vi "BaseProvider_DesignPattern_GetPatterns.vi"(1 "FilterOnProviders(Ignored If Empty)":string, 2 "FilterOnTemplate(Ignored If Empty)":string, 5 "error in (no error)":errorcluster) -> (15 "DesignPatterns":T1[](array[typedef]), 19 "error out":errorcluster)   [LabVIEW 2020]
uses:
  DesignPatternsData.ctl
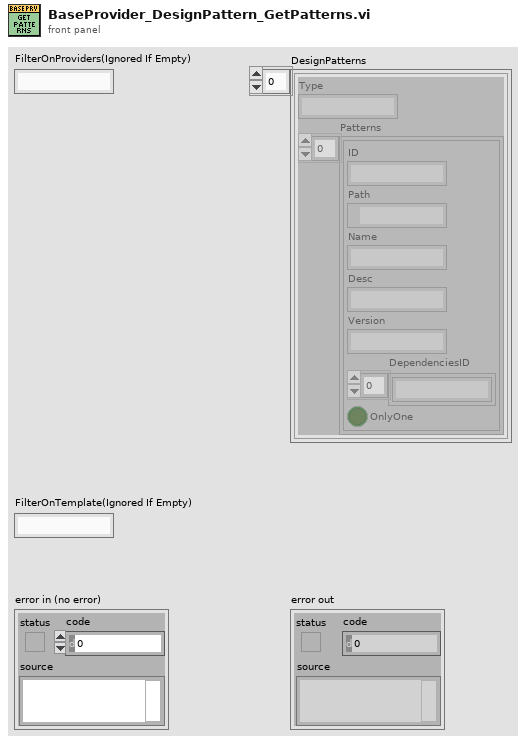
[diagram p1: front panel]
types:
  T1 = typedef "DesignPatternsData.ctl" = cluster{"Type":string, "Patterns":cluster{"ID":string, "Path":path, "Name":string, "Desc":string, "Version":string, "DependenciesID":string[], "OnlyOne":bool}[]}
  T2 = cluster{"Cancelled":bool, "IniFiles":path[], "IniFilesContent":cluster{"ID":string, "Version":string, "PlugIn":path, "Type":string, "Name":string, "Desc":string, "Supports":cluster{"Provider":string, "Templates":string}[], "DependenciesID":string[], "OnlyOne":bool}[], "DesignPatterns":T1[]}
  T3 = cluster{"ID":string, "Version":string, "PlugIn":path, "Type":string, "Name":string, "Desc":string, "Supports":cluster{"Provider":string, "Templates":string}[], "DependenciesID":string[], "OnlyOne":bool}[]
  T4 = cluster{"ID":string, "Version":string, "PlugIn":path, "Type":string, "Name":string, "Desc":string, "Supports":cluster{"Provider":string, "Templates":string}[], "DependenciesID":string[], "OnlyOne":bool}
  T5 = cluster{"ID":string, "Path":path, "Name":string, "Desc":string, "Version":string, "DependenciesID":string[], "OnlyOne":bool}[]
  T6 = cluster{"ID":string, "Path":path, "Name":string, "Desc":string, "Version":string, "DependenciesID":string[], "OnlyOne":bool}
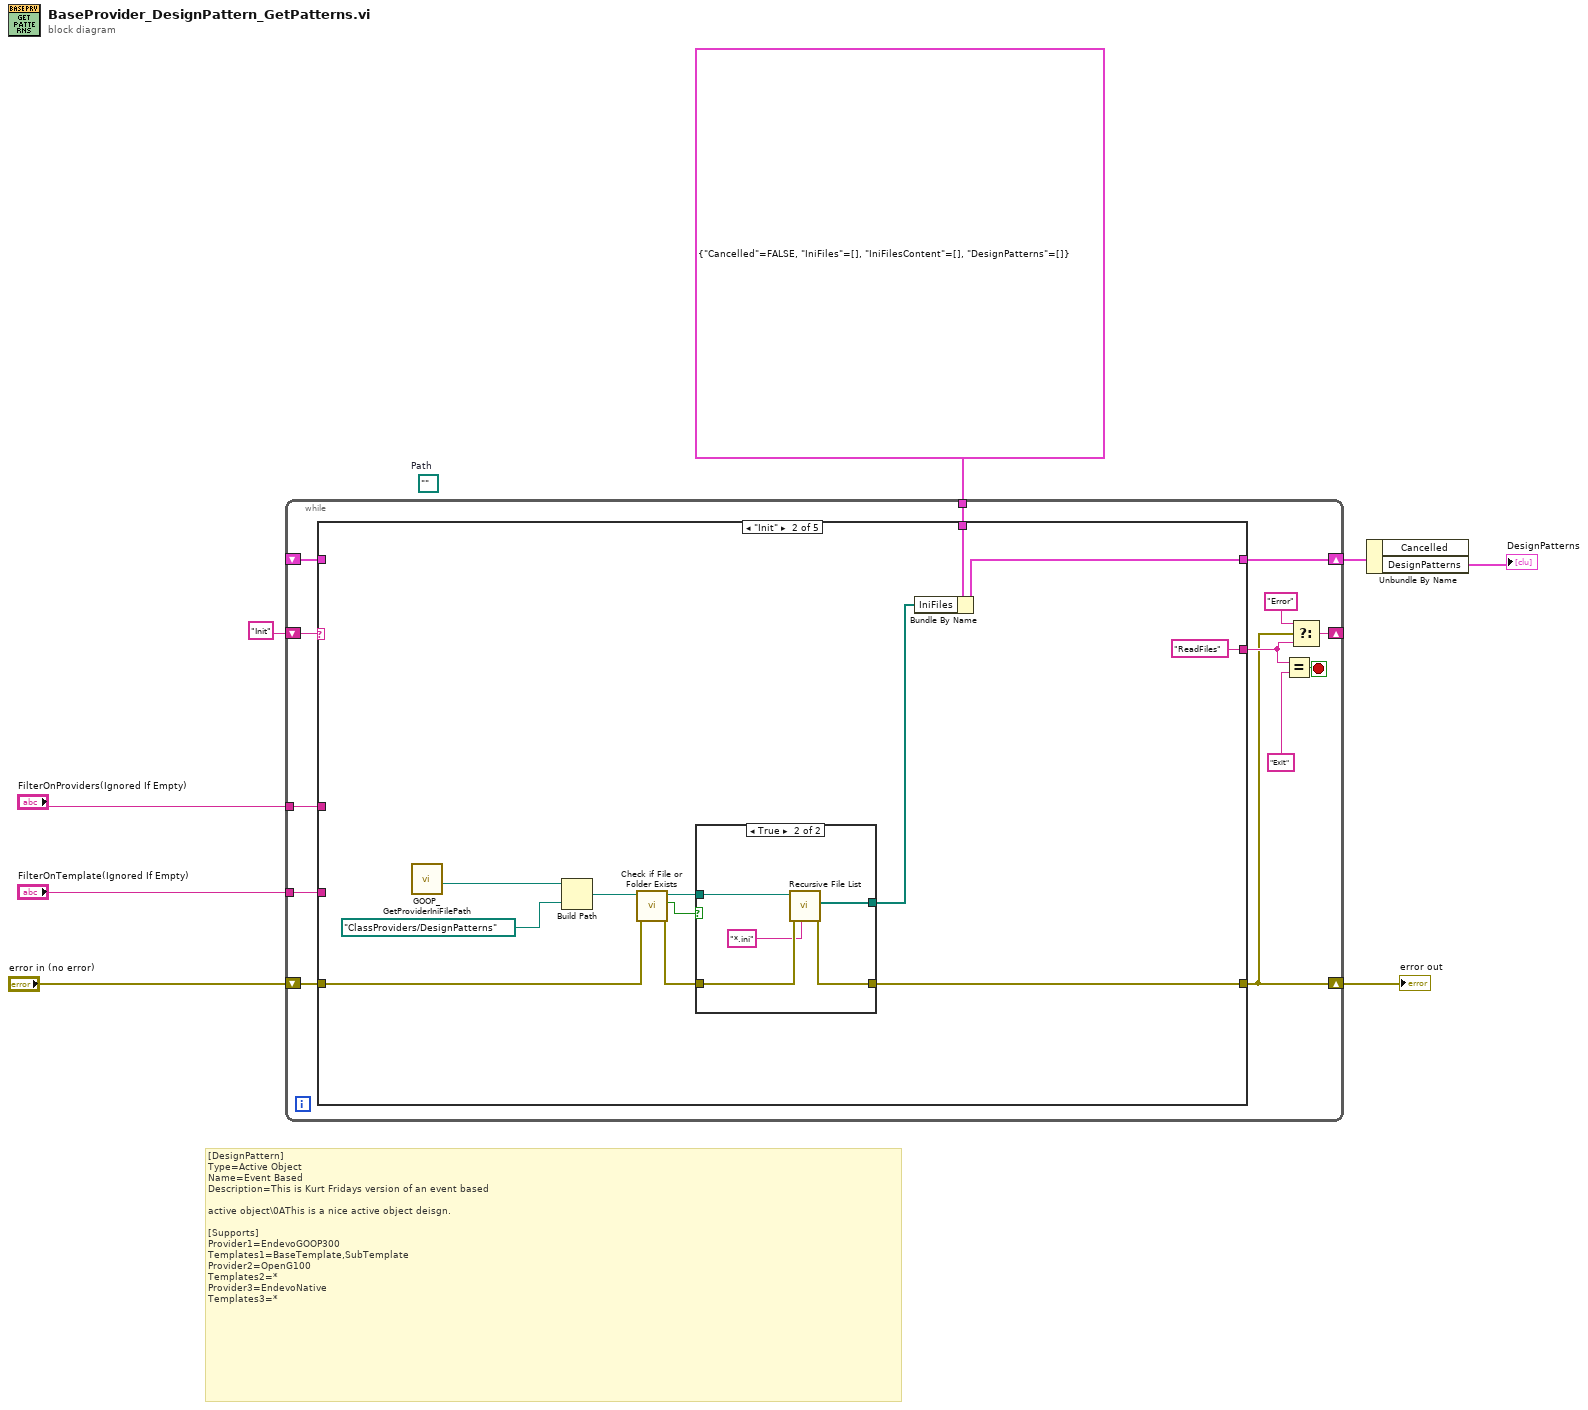
[diagram p0: block diagram]
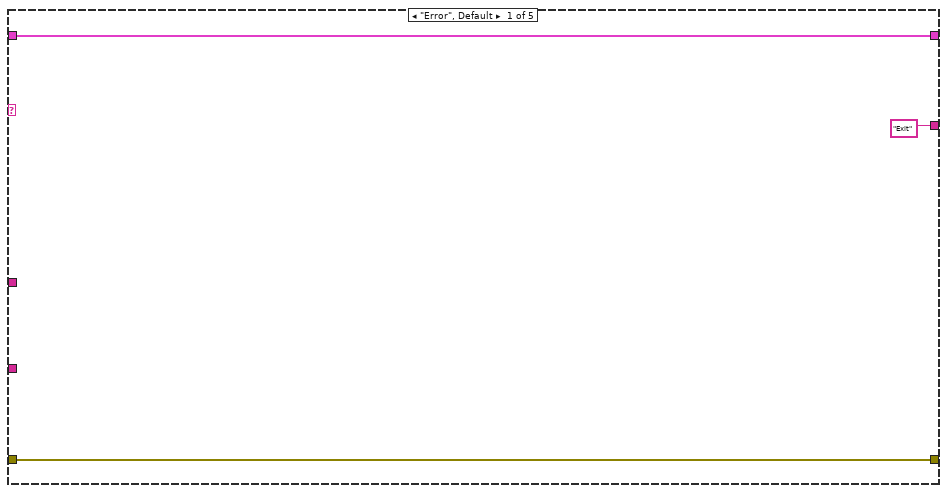
[diagram p2: hidden frame]
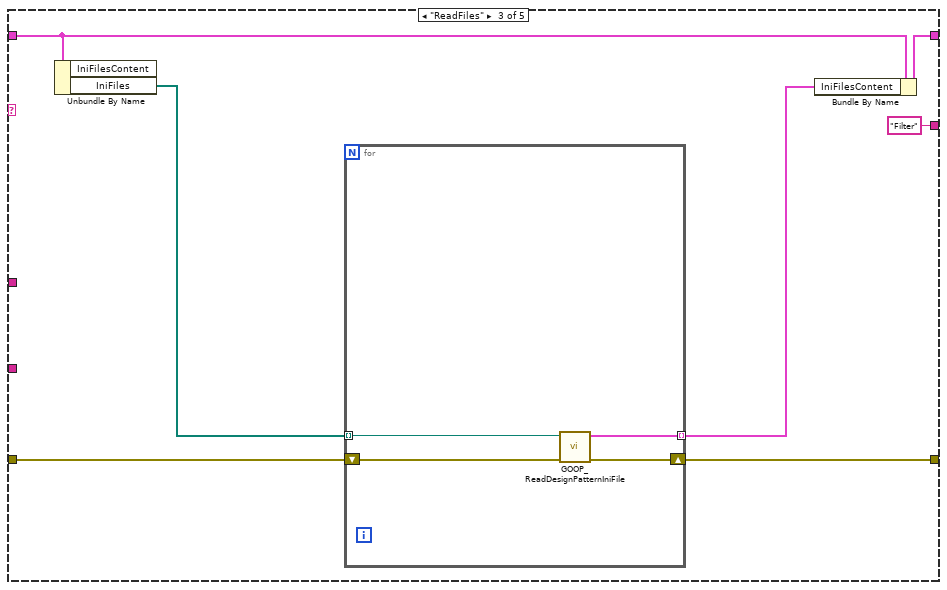
[diagram p4: hidden frame]
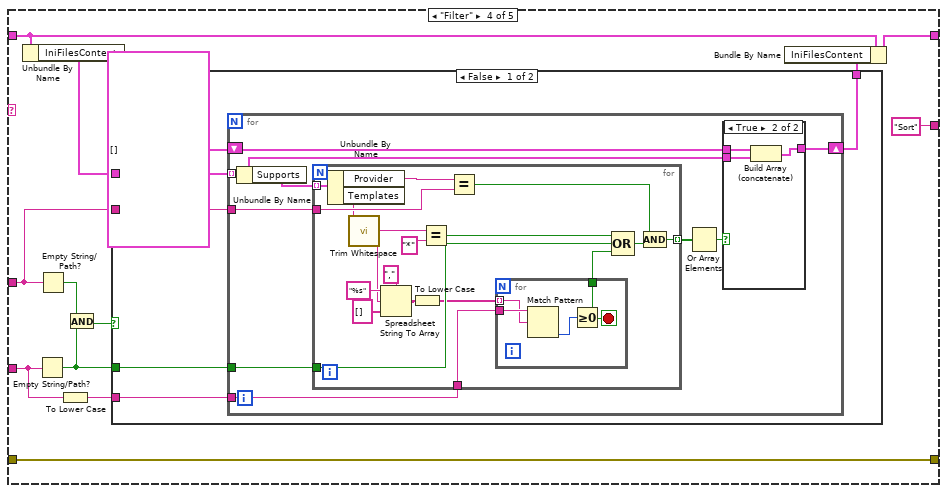
[diagram p5: hidden frame]
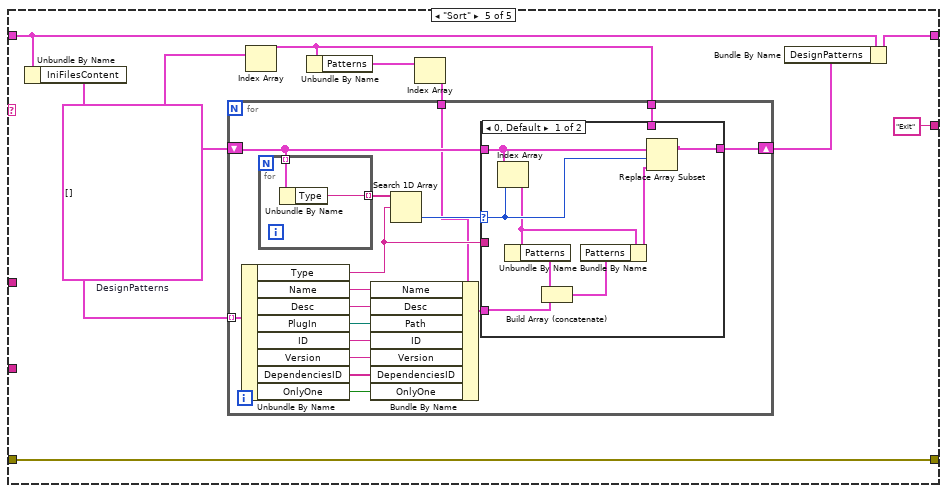
[diagram p8: hidden frame]
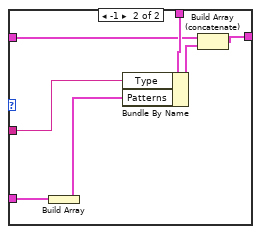
[diagram p9: hidden frame]
diagram:
  (unwired) path ""  # Path
  # "[DesignPattern]\nType=Active Object\nName=Event Based\nDescription=This is Kurt Fridays version of an event based \n\nactive object\\0AThis is a nice active object deisgn.\n\n[Supports]\nProvider1=EndevoGOOP300\nTemplates1=BaseTemplate,SubTemplate\nProvider2=OpenG100\nTemplates2=*\nProvider3=EndevoNative\nTemplates3=*"
  n1 = while {
    shift-right: [w14] -> w5
    shift-left: "error in (no error)" -> [w21]
    shift-right: [w19] -> _
    shift-left: "Init" -> [w20]
    shift-right: [w13] -> w7
    shift-left: _ -> [w12]
    tunnel: "FilterOnProviders(Ignored If Empty)" -> [w11]
    tunnel: "FilterOnTemplate(Ignored If Empty)" -> [w10]
    tunnel: T2 {"Cancelled"=FALSE, "IniFiles"=[], "IniFilesContent"=[], "DesignPatterns"=[]} -> [w9]
    stop <- w18 stop-if-true
    n2 = case shown="\"Init\"" w20 {
      tunnel: w21 -> [w24 w26 w48 w64 w116]
      tunnel: [w24 w32 w46 w64 w116] -> w14
      tunnel: ["Exit" "ReadFiles" "Filter" "Sort" "Exit"] -> w15
      tunnel: [w22 w35 w44 w59 w114] -> w13
      tunnel: w12 -> [w22 _ w45 w61 w115]
      tunnel: w11 -> [_ _ _ w57 _]
      tunnel: w10 -> [_ _ _ w55 _]
      tunnel: w9 -> [_ w30 _ _ _]
      frame "Error", Default {
      }
      frame "Init" {
        n3 = call "GOOP_GetProviderIniFilePath.vi"() -> ("ProviderMainFolder"=w34:path)  [unwired: 10 in, 1 out]
        n4 = Build Path(base path=w34, name or relative path=path "ClassProviders/DesignPatterns" ("base path")) -> (appended path=w29:path)
        n5 = call <vilib>:"Check if File or Folder Exists.vi"("error in (no error)"=w26, "path"=w29) -> ("error out"=w27:errorcluster, "file or folder exists?"=w25:bool, "dup path"=w28:path)  [unwired: 7 in]
        n6 = case shown="True" w25 {
          tunnel: w28 -> [_ w42]
          tunnel: w27 -> [w37 w41]
          tunnel: [w37 w40] -> w32
          tunnel: [_ w38] -> w31
          frame False {
          }
          frame True {
            n7 = call <vilib>:"Recursive File List.vi"("pattern"="*.ini", "error in (no error)"=w41, "Folder Path"=w42) -> ("error out"=w40:errorcluster, "All Files in Dir"=w38:path[])  [unwired: 4 in, 3 out]
          }
        }
        n8 = Bundle By Name(cluster=w30, "IniFiles"=w31) -> (w35:T2)
      }
      frame "ReadFiles" {
        n9 = Unbundle By Name(w45) -> ("IniFiles"=w47:path[])  [unwired: 1 out]
        n10 = for {
          shift-right: [w52] -> w46
          shift-left: w48 -> [w53]
          tunnel: w47 -> [w50] mode=indexing
          tunnel: [w51] -> w43 mode=indexing
          n11 = call "GOOP_ReadDesignPatternIniFile.vi"("error in (no error)"=w53, "Path"=w50) -> ("error out"=w52:errorcluster, "cluster"=w51:T4)  [unwired: 8 in]
        }
        n12 = Bundle By Name(cluster=w45, "IniFilesContent"=w43) -> (w44:T2)
      }
      frame "Filter" {
        n13 = Unbundle By Name(w61) -> ("IniFilesContent"=w65:T3)
        n14 = Empty String/Path?(string/path=w55) -> (empty?=w56:bool)
        n15 = Empty String/Path?(string/path=w57) -> (empty?=w63:bool)
        n16 = To Lower Case(string=w55) -> (all lower case string=w54:string)
        n17 = And(x=w63, y=w56) -> (x .and. y?=w62:bool)
        n18 = case shown="False" w62 {
          tunnel: w65 -> [w71 w107]
          tunnel: [w67 w107] -> w60
          tunnel: w57 -> [w70 _]
          tunnel: w54 -> [w69 _]
          tunnel: w56 -> [w68 _]
          frame False {
            n19 = for {
              tunnel: w71 -> [w73] mode=indexing
              shift-right: [w78] -> w67
              shift-left: T3 [] -> [w79]
              tunnel: w70 -> [w77]
              tunnel: w69 -> [w72]
              tunnel: w68 -> [w76]
              n20 = Unbundle By Name(w73) -> ("Supports"=w80:cluster{"Provider":string, "Templates":string}[])
              n21 = for {
                tunnel: w80 -> [w102] mode=indexing
                tunnel: w77 -> [w100]
                tunnel: w72 -> [w86]
                tunnel: w76 -> [w95]
                tunnel: [w93] -> w75 mode=indexing
                n22 = Unbundle By Name(w102) -> ("Provider"=w101:string, "Templates"=w92:string)
                n23 = call <vilib>:"Trim Whitespace.vi"("string"=w92) -> ("trimmed string"=w91:string)  [unwired: 1 in]
                n24 = Spreadsheet String To Array(delimiter (Tab)=",", format string="%s", spreadsheet string=w91, array type (2D Dbl)=string[] []) -> (array=w96:string[])
                n25 = To Lower Case(string=w96) -> (all lower case string=w87:string[])
                n26 = Equal?(x=w91, y="*" ("element")) -> (x = y?=w88:bool)
                n27 = Equal?(x=w101, y=w100) -> (x = y?=w89:bool)
                n28 = for {
                  tunnel: w87 -> [w103] mode=indexing
                  tunnel: w86 -> [w104]
                  tunnel: [w105] -> w85
                  stop <- w105 stop-if-true
                  n29 = Match Pattern(string=w104, regular expression=w103) -> (offset past match=w106:i32)  [unwired: 1 in, 3 out]
                  n30 = Greater Or Equal To 0?(x=w106) -> (x >= 0?=w105:bool)
                }
                n31 = Compound Arithmetic op=OR(w88, w95, w85) -> (w94:bool)
                n32 = Compound Arithmetic op=AND(w89, w94) -> (w93:bool)
              }
              n33 = Or Array Elements(Boolean array=w75) -> (logical OR=w74:bool)
              n34 = case shown="True" w74 {
                tunnel: w79 -> [w81 w84]
                tunnel: [w81 w83] -> w78
                tunnel: w73 -> [_ w82]
                frame False {
                }
                frame True {
                  n35 = Build Array (concatenate)(w84, w82) -> (w83:T3)
                }
              }
            }
          }
          frame True {
          }
        }
        n36 = Bundle By Name(cluster=w61, "IniFilesContent"=w60) -> (w59:T2)
      }
      frame "Sort" {
        w111 = T1[] []  # DesignPatterns
        n37 = Unbundle By Name(w115) -> ("IniFilesContent"=w117:T3)
        n38 = Index Array(array=w111) -> (element=w110:T1)  [unwired: 1 in]
        n39 = Unbundle By Name(w110) -> ("Patterns"=w109:T5)
        n40 = Index Array(array=w109) -> (element=w108:T6)  [unwired: 1 in]
        n41 = for {
          tunnel: w117 -> [w132] mode=indexing
          shift-right: [w133] -> w112
          shift-left: w111 -> [w131]
          tunnel: w110 -> [w128]
          tunnel: w108 -> [w123]
          n42 = Unbundle By Name(w132) -> ("Type"=w127:string, "Name"=w126:string, "Desc"=w125:string, "PlugIn"=w124:path, "ID"=w121:string, "Version"=w120:string, "DependenciesID"=w119:string[], "OnlyOne"=w118:bool)
          n43 = for {
            tunnel: w131 -> [w135] mode=indexing
            tunnel: [w134] -> w130 mode=indexing
            n44 = Unbundle By Name(w135) -> ("Type"=w134:string)
          }
          n45 = Bundle By Name(cluster=w123, "Name"=w126, "Desc"=w125, "Path"=w124, "ID"=w121, "Version"=w120, "DependenciesID"=w119, "OnlyOne"=w118) -> (w122:T6)
          n46 = Search 1D Array(1D array=w130, element=w127) -> (index of element=w129:i32)  [unwired: 1 in]
          n47 = case shown="0, Default" w129 {
            selector: w129 -> [w142 _]
            tunnel: w131 -> [w143 w144]
            tunnel: [w136 w150] -> w133
            tunnel: w128 -> [_ w149]
            tunnel: w127 -> [_ w145]
            tunnel: w122 -> [w139 w146]
            frame 0, Default {
              n48 = Index Array(array=w143, index=w142) -> (element=w141:T1)
              n49 = Unbundle By Name(w141) -> ("Patterns"=w140:T5)
              n50 = Build Array (concatenate)(w140, w139) -> (w138:T5)
              n51 = Bundle By Name(cluster=w141, "Patterns"=w138) -> (w137:T1)
              n52 = Replace Array Subset(array=w143, new element=w137, index=w142) -> (w136:T1[])
            }
            frame -1 {
              n53 = Build Array(w146) -> (w147:T5)
              n54 = Bundle By Name(cluster=w149, "Type"=w145, "Patterns"=w147) -> (w148:T1)
              n55 = Build Array (concatenate)(w144, w148) -> (w150:T1[])
            }
          }
        }
        n56 = Bundle By Name(cluster=w115, "DesignPatterns"=w112) -> (w114:T2)
      }
    }
    n57 = Equal?(x=w15, y="Exit") -> (x = y?=w18:bool)
    n58 = Select(t="Error", s=w14, f=w15) -> (s? t:f=w19:string)
  }
  "error out" <- w5
  n59 = Unbundle By Name(w7) -> ("DesignPatterns"=→"DesignPatterns":T1[])  [unwired: 1 out]
